vi "example test.vi"() -> (0 "input lookup error":errorcluster, 1 "init error":errorcluster, 2 "correct execution settings":bool, 3 "output lookup error":errorcluster, 4 "input error":errorcluster, 5 "serialization problem":errorcluster, 6 "no data written":bool, 7 "invalid configuration":errorcluster, 8 "final error":errorcluster, 9 "output error":errorcluster)   [LabVIEW 2014, in "SQLite tests.lvlib"]
doc: "This VI shows an example for how to test the Runtime functionality of the module. This will need to be modified according to module functionality."
uses:
  SQLite tests.lvlib
  module/configuration/SQLite configuration.lvclass
  <vilib>/NI/Tag Bus Module Framework/channel/channel classification.ctl
  <vilib>/NI/Tag Bus/tag/Data Type.ctl
  module/execution/SQLite runtime.lvclass
  <vilib>/NI/Tag Bus/dictionary/data dictionary.lvclass/data dictionary.ctl
  <vilib>/NI/Tag Bus/dictionary/lookup polymorphs/locate double.vi
  <vilib>/NI/Tag Bus/table/data polymorphs/write one/write Double.vi
  <vilib>/NI/Tag Bus/table/data polymorphs/read one/read Double.vi
  <vilib>/NI/Tag Bus/dictionary/search/find data index.vi
  <vilib>/NI/Tag Bus/dictionary/search/search string list.vi
  <vilib>/NI/Tag Bus/dictionary/tag not found.vi
  <vilib>/NI/Tag Bus/dictionary/data dictionary.lvclass
  <vilib>/NI/Tag Bus/table/data table.lvlib
  <vilib>/NI/Tag Bus Module Framework/channel/TBM channel.lvclass
  <vilib>/NI/Tag Bus/tag/tag descriptor.lvclass
  <vilib>/NI/Configuration Framework/serializable configuration/NISE_CEF_serializable configuration.lvclass
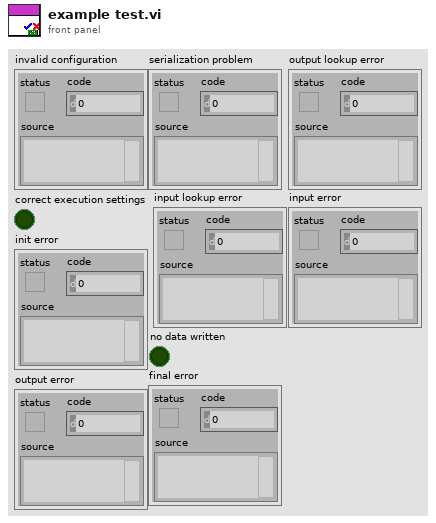
[diagram p1: front panel]
types:
  T1 = typedef "TBM channel.lvclass/channel classification.ctl" = enum16{"input data", "output data", "processing parameter", "processing result"}
  T2 = typedef "tag bus.lvlib/tag descriptor.lvclass/Data Type.ctl" = enum16{"Double", "Single", "I64", "I32", "I16", "I8", "U64", "U32", "U16", "U8", "Boolean", "String", "Array of Double", "Array of Single", "Array of I64", "Array of I32", "Array of I16", "Array of I8", "Array of U64", "Array of U32", "Array of U16", "Array of U8", "Array of Boolean", "Array of String"}
  T3 = cluster{"channel":refnum<class "TBM channel.lvclass">}
  T4 = typedef "TBM channel.lvclass/data tables.ctl" = cluster{"input data":T5, "processing parameter":T5, "processing result":T5, "output data":T5}
  T5 = typedef "tag bus.lvlib/dictionary table pair.ctl" = cluster{"data dictionary":refnum<class "data dictionary.lvclass">, "data table":T6}
  T6 = typedef "tag bus.lvlib/data table.lvlib/data table.ctl" = cluster{"Double":dbl[], "Single":sgl[], "I64":i64[], "I32":i32[], "I16":i16[], "I8":i8[], "U64":u64[], "U32":u32[], "U16":u16[], "U8":u8[], "Boolean":bool[], "String":string[], "Array of Double":cluster{"DBL Array":dbl[]}[], "Array of Single":cluster{"SGL Array":sgl[]}[], "Array of I64":cluster{"I64 Array":i64[]}[], "Array of I32":cluster{"I32 Array":i32[]}[], "Array of I16":cluster{"I16 Array":i16[]}[], "Array of I8":cluster{"I8 Array":i8[]}[], "Array of U64":cluster{"U64 Array":u64[]}[], "Array of U32":cluster{"U32 Array":u32[]}[], "Array of U16":cluster{"U16 Array":u16[]}[], "Array of U8":cluster{"U8 Array":u8[]}[], "Array of Boolean":cluster{"Boolean Array":bool[]}[], "Array of String":cluster{"String Array":string[]}[]}
  T7 = typedef "TBM module execution interface.lvclass/execution settings.ctl" = cluster{"reads inputs":bool, "processes data":bool, "writes outputs":bool}
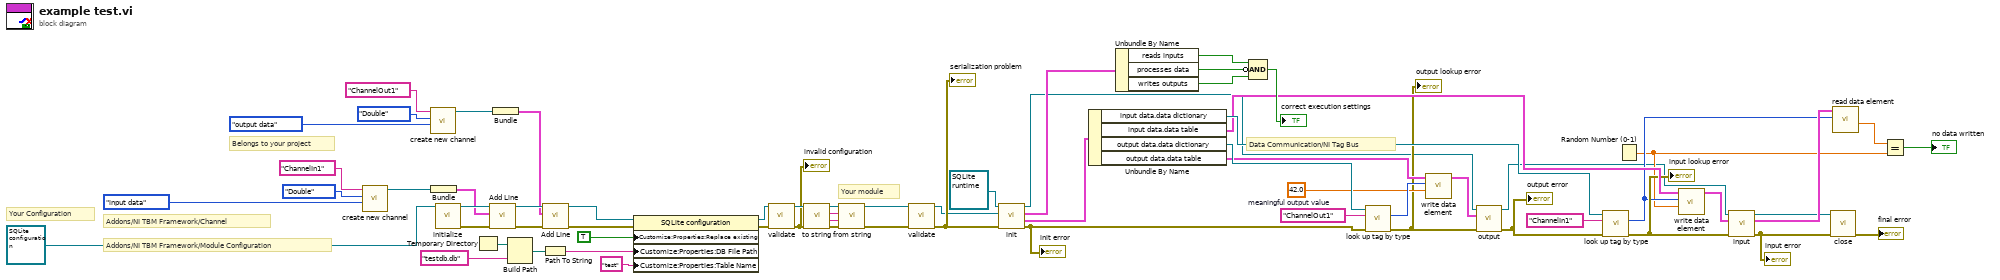
[diagram p0: block diagram]
diagram:
  w29 = 42.0  # meaningful output value
  # "Data Communication/NI Tag Bus"
  # "Your module"
  # "Your Configuration"
  # "Addons/NI TBM Framework/Module Configuration"
  # "Belongs to your project"
  # "Addons/NI TBM Framework/Channel"
  n1 = call <vilib>:"create new channel.vi"("channel classification"=channel_classification."input data", "data type"=Data_Type."Double", "channel name"="ChannelIn1") -> ("channel"=w20:refnum<class "TBM channel.lvclass">)  [unwired: 8 in]
  n2 = call <vilib>:"create new channel.vi"("channel classification"=channel_classification."output data", "data type"=Data_Type."Double", "channel name"="ChannelOut1") -> ("channel"=w18:refnum<class "TBM channel.lvclass">)  [unwired: 8 in]
  n3 = Bundle("channel"=w20) -> (w19:T3)  [unwired: 1 in]
  n4 = call <vilib>:"initialize.vi"("configuration in"=refnum<class "SQLite configuration.lvclass"> refnum ("tag bus configurable plugin module configuration")) -> ("error out"=w21:errorcluster, "configuration out"=w22:refnum<class "SQLite configuration.lvclass">)  [unwired: 8 in, 1 out]
  n5 = Temporary Directory() -> (w14:path)
  n6 = call "Add Line.vi"("error in"=w21, "Line"=w19, "SQLite configuration in"=w22) -> ("error out"=w23:errorcluster, "SQLite configuration out"=w24:refnum<class "SQLite configuration.lvclass">)  [unwired: 6 in, 1 out]
  n7 = Bundle("channel"=w18) -> (w17:T3)  [unwired: 1 in]
  n8 = Build Path(base path=w14, name or relative path="testdb.db") -> (appended path=w11:path)
  n9 = Path To String(path=w11) -> (string=w2:string)
  n10 = call "Add Line.vi"("error in"=w23, "Line"=w17, "SQLite configuration in"=w24) -> ("error out"=w9:errorcluster, "SQLite configuration out"=w16:refnum<class "SQLite configuration.lvclass">)  [unwired: 6 in, 1 out]
  n11 = property class="SQLite configuration"(reference=w16, error in=w9, "Customize:Properties:Replace existing"=TRUE ("Replace existing"), "Customize:Properties:DB File Path"=w2, "Customize:Properties:Table Name"="test" ("Table Name")) -> (reference out=w10:refnum<class "SQLite configuration.lvclass">, error out=w8:errorcluster)
  n12 = call-dynamic "validate.vi"("error in"=w8, "SQLite configuration in"=w10) -> ("error out"=w59:errorcluster, "SQLite configuration out"=w60:refnum<class "SQLite configuration.lvclass">)  [unwired: 8 in]
  "invalid configuration" <- w59
  n13 = call-dynamic "to string.vi"("error in"=w59, "SQLite configuration in"=w60) -> ("error out"=w55:errorcluster, "data"=w56:string, "version"=w57:string, "SQLite configuration out"=w58:refnum<class "SQLite configuration.lvclass">)  [unwired: 6 in]
  n14 = call-dynamic "from string.vi"("error in"=w55, "data"=w56, "version"=w57, "SQLite configuration in"=w58) -> ("error out"=w53:errorcluster, "SQLite configuration out"=w54:refnum<class "SQLite configuration.lvclass">)  [unwired: 6 in]
  n15 = call-dynamic "validate.vi"("error in"=w53, "SQLite configuration in"=w54) -> ("error out"=w51:errorcluster, "SQLite configuration out"=w50:refnum<class "SQLite configuration.lvclass">)  [unwired: 8 in]
  "serialization problem" <- w51
  n16 = call-dynamic "init.vi"("error in"=w51, "TBM module configuration in"=w50, "SQLite runtime in"=refnum<class "SQLite runtime.lvclass"> refnum ("tag bus configurable plugin module")) -> ("error out"=w1:errorcluster, "data allocations"=w44:T4, "execution settings"=w49:T7, "SQLite runtime out"=w7:refnum<class "SQLite runtime.lvclass">)  [unwired: 5 in]
  "init error" <- w1
  n17 = Unbundle By Name(w44) -> ("input data.data dictionary"=w43:refnum<class "data dictionary.lvclass">, "input data.data table"=w41:T6, "output data.data dictionary"=w33:refnum<class "data dictionary.lvclass">, "output data.data table"=w30:T6)
  n18 = Unbundle By Name(w49) -> ("reads inputs"=w46:bool, "processes data"=w48:bool, "writes outputs"=w47:bool)
  n19 = Compound Arithmetic op=AND(w46, invert w48, w47) -> (→"correct execution settings":bool)
  n20 = call-poly <vilib>:"look up tag by type.vi"("error in"=w1, "name"="ChannelOut1" ("channel name"), "data dictionary in"=w33) -> ("error out"=w28:errorcluster, "index"=w31:i32)  [unwired: 6 in, 1 out]
  "output lookup error" <- w28
  n21 = call-poly <vilib>:"write data element.vi"("value"=w29, "index"=w31, "data table in"=w30) -> ("data table out"=w27:T6)  [unwired: 8 in]
  n22 = call-dynamic "output.vi"("error in"=w28, "data table in"=w27, "SQLite runtime in"=w7) -> ("error out"=w3:errorcluster, "SQLite runtime out"=w6:refnum<class "SQLite runtime.lvclass">)  [unwired: 6 in, 1 out]
  "output error" <- w3
  n23 = call-poly <vilib>:"look up tag by type.vi"("error in"=w3, "name"="ChannelIn1" ("channel name"), "data dictionary in"=w43) -> ("error out"=w40:errorcluster, "index"=w37:i32)  [unwired: 6 in, 1 out]
  "input lookup error" <- w40
  n24 = Random Number (0-1)() -> (number: 0 to 1=w36:dbl)
  n25 = call-poly <vilib>:"write data element.vi"("value"=w36, "index"=w37, "data table in"=w41) -> ("data table out"=w39:T6)  [unwired: 8 in]
  n26 = call-dynamic "input.vi"("error in"=w40, "data table in"=w39, "SQLite runtime in"=w6) -> ("error out"=w4:errorcluster, "data table out"=w38:T6, "SQLite runtime out"=w5:refnum<class "SQLite runtime.lvclass">)  [unwired: 6 in]
  "input error" <- w4
  n27 = call-dynamic "close.vi"("error in"=w4, "SQLite runtime in"=w5) -> ("error out"=→"final error":errorcluster)  [unwired: 9 in]
  n28 = call-poly <vilib>:"read data element.vi"("index"=w37, "data table in"=w38) -> ("value"=w35:dbl)  [unwired: 8 in, 1 out]
  n29 = Equal?(x=w35, y=w36) -> (x = y?=→"no data written":bool)
